vi "libssh2_channel_get_exit_signal.vi"(8 "error in (no error)":errorcluster, 11 "channel":T1) -> (0 "error out":errorcluster, 1 "errmsg":string, 2 "exitsignal":string, 4 "langtag":string)   [LabVIEW 2017, in "libssh2.lvlib"]
doc: "Get the exit signal from a channel."
uses:
  libssh2.lvlib
  Channel Refnum.ctl
  Acquire Session.vi
  Release Session.vi
  Not A Channel.vi
  <vilib>/Utility/error.llb/Error Cluster From Error Code.vi
  Global Settings.vi
  Read Channel Refnum.vi
  Read Session Refnum.vi
  <vilib>/Utility/semaphor.llb/Acquire Semaphore.vi
  <vilib>/Utility/semaphor.llb/Release Semaphore.vi
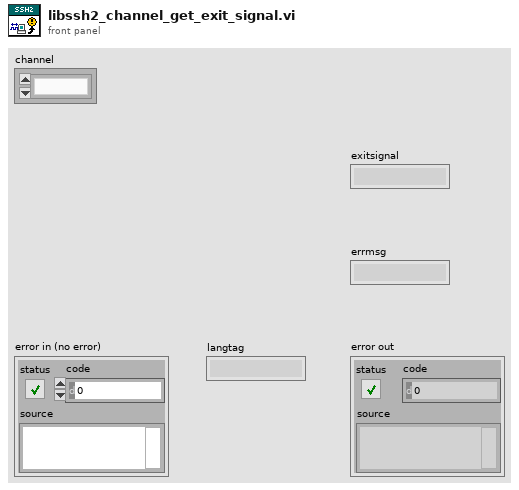
[diagram p1: front panel]
types:
  T1 = typedef "libssh2.lvlib/Channel Refnum.ctl" = refnum<k1>
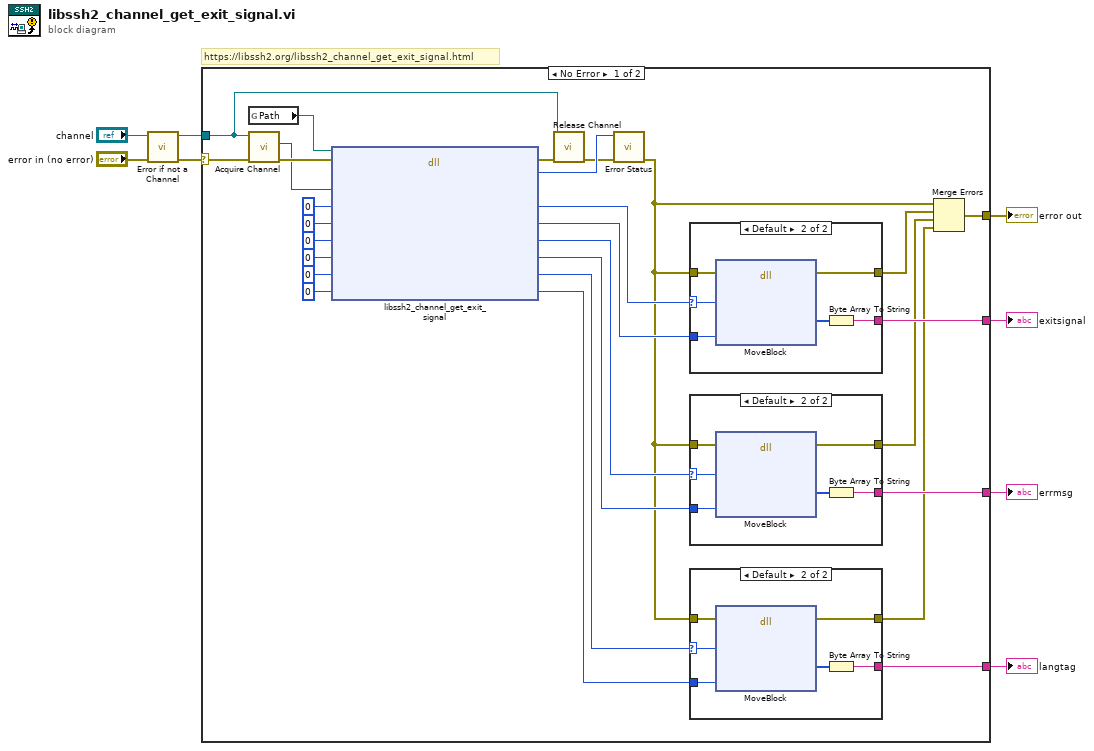
[diagram p0: block diagram]
diagram:
  # "https://libssh2.org/libssh2_channel_get_exit_signal.html"
  n1 = call "Error if not a Channel.vi"("error in (no error)"="error in (no error)", "channel"="channel") -> ("error out"=w3:errorcluster, "channel out"=w1:T1)  [unwired: 8 in]
  n2 = case shown="No Error" w3 {
    selector: w3 -> [w14 w58]
    tunnel: [w33 _] -> w8
    tunnel: w1 -> [w9 _]
    tunnel: [w25 w58] -> w7
    tunnel: [w21 _] -> w6
    tunnel: [w16 _] -> w5
    frame No Error {
      n3 = global read "Global Settings.vi" "Path"() -> (w13:path)
      n4 = call "Acquire Channel.vi"("error in (no error)"=w14, "channel"=w9) -> ("error out"=w28:errorcluster, "LIBSSH2_CHANNEL*"=w27:u64)  [unwired: 8 in]
      n5 = dll-call lib="?" fn="libssh2_channel_get_exit_signal"(path in=w13, error in=w28, "channel"=w27, "exitsignal"=u64 0, "exitsignal_len"=u64 0, "errmsg"=u64 0, "errmsg_len"=u64 0, "langtag"=u64 0, "langtag_len"=u64 0) -> (error out=w19:errorcluster, "return value"=w11:i32, "exitsignal"=w24:u64, "exitsignal_len"=w32:u64, "errmsg"=w23:u64, "errmsg_len"=w22:u64, "langtag"=w18:u64, "langtag_len"=w17:u64)  [unwired: 2 in, 1 out]
      n6 = call "Release Channel.vi"("error in (no error)"=w19, "channel"=w9) -> ("error out"=w10:errorcluster)  [unwired: 9 in]
      n7 = call "Error Status.vi"("error in (no error)"=w10, "return value"=w11) -> ("error out"=w12:errorcluster)  [unwired: 8 in, 1 out]
      n8 = case shown="Default" w24 {
        selector: w24 -> [_ w52]
        tunnel: [_ w56] -> w33
        tunnel: w32 -> [_ w55]
        tunnel: [w51 w54] -> w26
        tunnel: w12 -> [w51 w53]
        frame 0 {
        }
        frame Default {
          n9 = dll-call lib="LabVIEW" fn="MoveBlock"(error in=w53, "ps"=w52, "size"=w55) -> (error out=w54:errorcluster, "pd"=w57:u8[])  [unwired: 6 in, 1 out]
          n10 = Byte Array To String(unsigned byte array=w57) -> (string=w56:string)
        }
      }
      n11 = case shown="Default" w23 {
        selector: w23 -> [_ w45]
        tunnel: [_ w49] -> w21
        tunnel: w22 -> [_ w48]
        tunnel: [w44 w47] -> w20
        tunnel: w12 -> [w44 w46]
        frame 0 {
        }
        frame Default {
          n12 = dll-call lib="LabVIEW" fn="MoveBlock"(error in=w46, "ps"=w45, "size"=w48) -> (error out=w47:errorcluster, "pd"=w50:u8[])  [unwired: 6 in, 1 out]
          n13 = Byte Array To String(unsigned byte array=w50) -> (string=w49:string)
        }
      }
      n14 = case shown="Default" w18 {
        selector: w18 -> [_ w38]
        tunnel: [_ w42] -> w16
        tunnel: w17 -> [_ w41]
        tunnel: [w37 w40] -> w15
        tunnel: w12 -> [w37 w39]
        frame 0 {
        }
        frame Default {
          n15 = dll-call lib="LabVIEW" fn="MoveBlock"(error in=w39, "ps"=w38, "size"=w41) -> (error out=w40:errorcluster, "pd"=w43:u8[])  [unwired: 6 in, 1 out]
          n16 = Byte Array To String(unsigned byte array=w43) -> (string=w42:string)
        }
      }
      n17 = Merge Errors(w12, w26, w20, w15) -> (w25:errorcluster)
    }
    frame Error {
    }
  }
  "error out" <- w7
  "exitsignal" <- w8
  "errmsg" <- w6
  "langtag" <- w5
